vi "Read I8.vi"(8 "error in (no error)":errorcluster, 11 "Event in":refnum<class "Event I8.lvclass">) -> (0 "error out":errorcluster, 2 "I8":i8, 3 "Event out":refnum<class "Event I8.lvclass">)   [LabVIEW 2023, in "MVC Actors.lvlib" / "Event I8.lvclass"]
uses:
  Event I8.lvclass
  Event I8.lvclass/Event I8.ctl
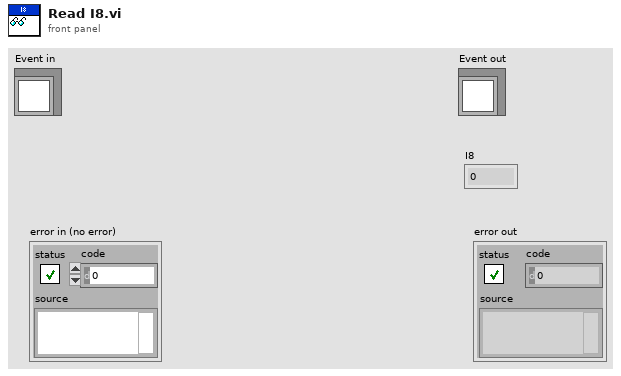
[diagram p1: front panel]
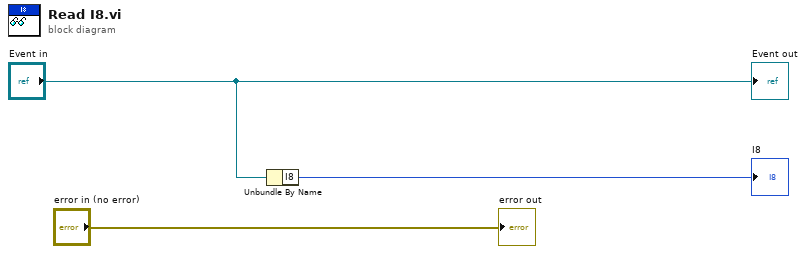
[diagram p0: block diagram]
diagram:
  n1 = Unbundle By Name("Event in") -> ("I8"=→"I8":i8)
  "Event out" <- "Event in"
  "error out" <- "error in (no error)"
